vi "wait ms.vi"(8 "error in":errorcluster, 10 "ms (1000)":dbl=1000.0) -> (0 "error out":errorcluster)   [LabVIEW 2025]
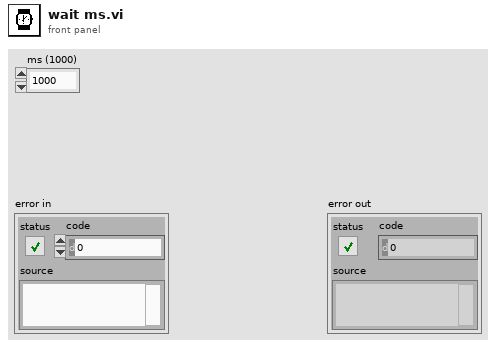
[diagram p1: front panel]
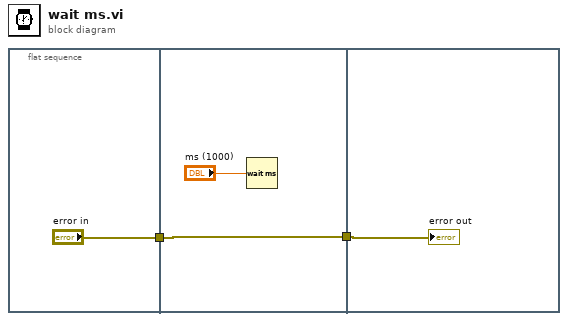
[diagram p0: block diagram]
diagram:
  n1 = flat-sequence {
    tunnel: ["error in"] -> w2
    tunnel: w2 -> [w4]
    tunnel: [w4] -> w1
    tunnel: w1 -> [w6]
    frame #0 {
    }
    frame #1 {
      n2 = Wait (ms)(milliseconds to wait="ms (1000)") -> ()  [unwired: 1 out]
    }
    frame #2 {
      "error out" <- w6
    }
  }
